vi "串口文本1.vi"() -> ()   [LabVIEW 2023]
uses:
  <vilib>/Instr/_visa.llb/VISA Configure Serial Port (Instr).vi
panel:
  out "报警":bool
  out "?":dbl
  out "重量":dbl(knob) scale=0.0..500.0
  in  "baud rate (9600)":u32=9600 caption="波特率"
  in  "最高阈值":dbl
  in  "停止":bool
  in  "端口":refnum<visa-resource-name>
  # "Labview电子秤显示界面"
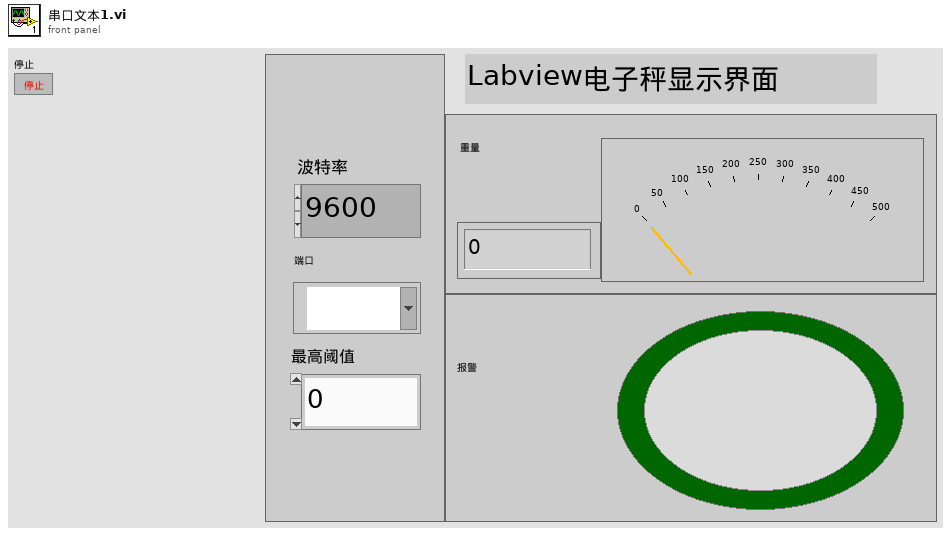
[diagram p1: front panel]
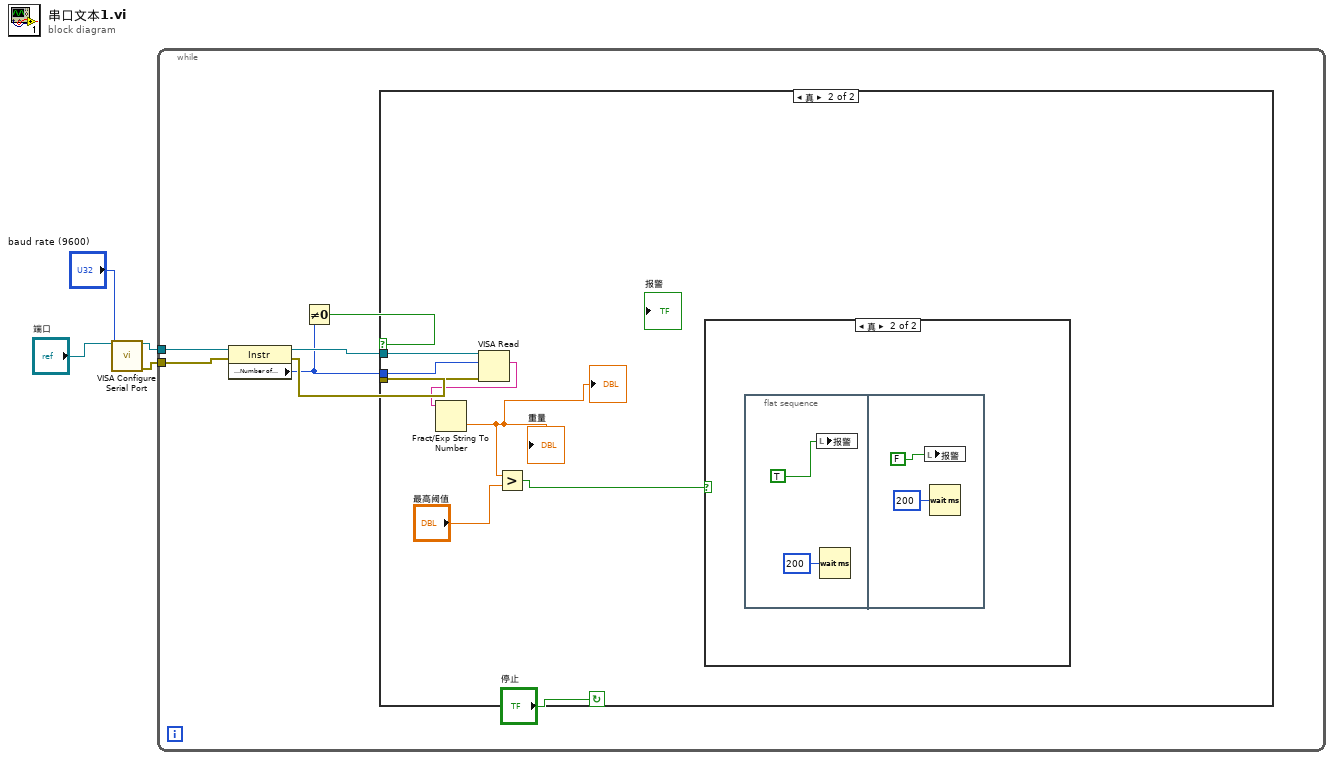
[diagram p0: block diagram]
diagram:
  n1 = call-poly "VISA Configure Serial Port"("VISA resource name"="端口", "baud rate (9600)"="baud rate (9600)") -> ("VISA resource name out"=w3:refnum<visa-resource-name>, "error out"=w2:errorcluster)  [unwired: 12 in]
  n2 = while {
    tunnel: w3 -> [w11]
    tunnel: w2 -> [w10]
    stop <- "停止" continue-if-true
    n3 = property class="Instr"(reference=w11, error in=w10) -> (reference out=w9:refnum<visa-resource-name>, error out=w8:errorcluster, "Serial Settings:Number of Bytes at Serial Port"=w7:u32)
    n4 = Not Equal To 0?(x=w7) -> (x != 0?=w6:bool)
    n5 = case shown="真" w6 {
      tunnel: w9 -> [_ w18]
      tunnel: w8 -> [_ w17]
      tunnel: w7 -> [_ w16]
      frame False {
      }
      frame True {
        n6 = VISA Read(VISA resource name=w18, byte count=w16, error in (no error)=w17) -> (read buffer=w14:string)  [unwired: 3 out]
        n7 = Fract/Exp String To Number(string=w14) -> (number=w13:dbl)  [unwired: 3 in, 1 out]
        "重量" <- w13
        "?" <- w13
        n8 = Greater?(x=w13, y="最高阈值") -> (0:w12:bool)
        n9 = case shown="真" w12 {
          frame False {
          }
          frame True {
            n10 = flat-sequence {
              frame #0 {
                n11 = local write "报警"(TRUE) -> ()
                n12 = Wait (ms)(milliseconds to wait=u32 200 ("等待时间（毫秒）")) -> ()  [unwired: 1 out]
              }
              frame #1 {
                n13 = local write "报警"(FALSE) -> ()
                n14 = Wait (ms)(milliseconds to wait=u32 200 ("等待时间（毫秒）")) -> ()  [unwired: 1 out]
              }
            }
          }
        }
      }
    }
  }
